vi "Release_Message_Queue.vi"(8 "error in (no error)":errorcluster={"status"=FALSE, "code"=0, "source"="\"\""}, 11 "Message Queue":refnum<queue>) -> (0 "error out":errorcluster)   [LabVIEW 2026]
doc: "Release queue refnum."
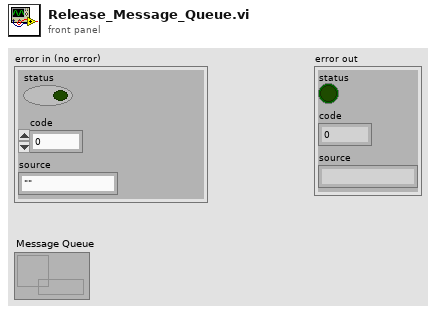
[diagram p1: front panel]
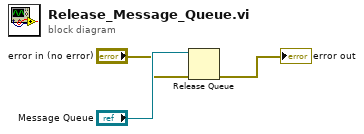
[diagram p0: block diagram]
diagram:
  n1 = Release Queue(queue="Message Queue", error in (no error)="error in (no error)") -> (error out=→"error out":errorcluster)  [unwired: 1 in, 2 out]
